vi "Delete Scale.vi"(8 "error in":errorcluster, 10 "Index":i32, 11 "references":T1) -> (0 "error out":errorcluster)   [LabVIEW 2014, in "Scaling editor node.lvclass"]
uses:
  Scaling editor node.lvclass
  <vilib>/NI/DCAF/Tag Editor Core/Table API/Table Manager/object ref.ctl
  <vilib>/NI/DCAF/Tag Editor Core/Configuration Editor/Classes/Engine Parent/Engine Parent Editor Node.lvclass
  <vilib>/NI/DCAF/Tag Editor Core/Configuration Editor/Classes/Module editor node/module editor node.lvclass
  module/configuration/Scaling configuration.lvclass
  <vilib>/NI/Configuration Framework/serializable configuration/NISE_CEF_serializable configuration.lvclass/NISE_CEF_serializable configuration.ctl
  <vilib>/Utility/LVClass/Get LV Class Name.vi
  <vilib>/NI/Configuration Framework/error generator/NISE_error generator.vi
  <vilib>/NI/Tag Bus Module Framework/channel/TBM channel.lvclass
  <vilib>/NI/Configuration Framework/serializable configuration/NISE_CEF_serializable configuration.lvclass
  <vilib>/NI/Module Execution Interface/Engine Configuration/engine configuration.lvclass
  <vilib>/NI/DCAF/Tag Editor Core/Table API/Table Manager/Table Manager.lvclass
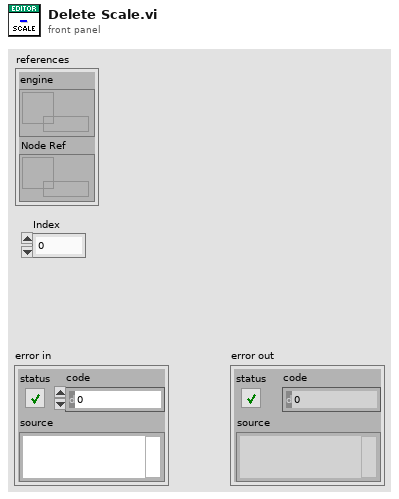
[diagram p1: front panel]
types:
  T1 = typedef "Table Manager.lvlib/Table Manager.lvclass/object ref.ctl" = cluster{"engine":refnum<data-value>, "Node Ref":refnum<data-value>}
  T2 = typedef "Scaling configuration.lvclass/scale data types.ctl" = enum16{"Double", "Single", "I64", "I32", "I16", "I8", "U64", "U32", "U16", "U8", "Boolean"}
  T3 = cluster{"input channel":refnum<class "TBM channel.lvclass">, "output channel":refnum<class "TBM channel.lvclass">, "input data type":T2, "output data type":T2}[]
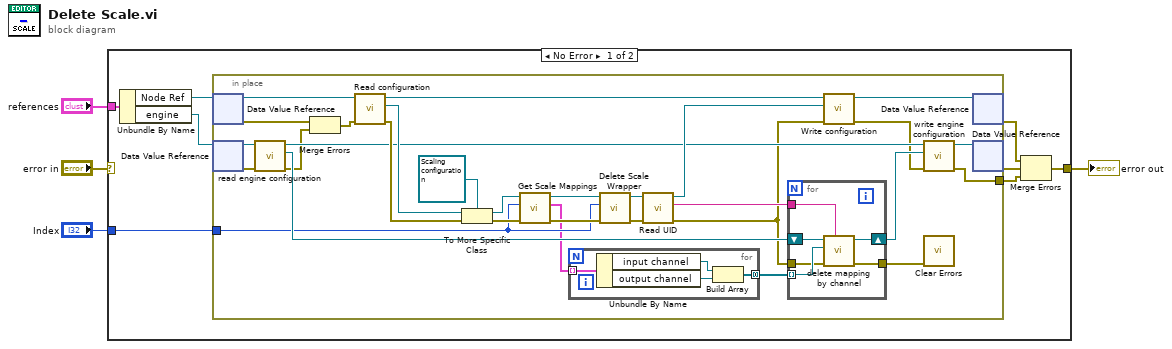
[diagram p0: block diagram]
diagram:
  n1 = case shown="No Error" "error in" {
    selector: "error in" -> [_ w53]
    tunnel: [w6 w53] -> w2
    tunnel: "Index" -> [w11 _]
    tunnel: "references" -> [w5 _]
    frame No Error {
      n2 = Unbundle By Name(w5) -> ("Node Ref"=w12:refnum<data-value>, "engine"=w10:refnum<data-value>)
      n3 = in-place {
        in-place-border: [w14] -> w7
        in-place-border: w11 -> [w19]
        n4 = in-place-dvr #1(w12) -> (w41:refnum<class "module editor node.lvclass">, w26:errorcluster)
        n5 = in-place-dvr #2(w10) -> (w36:refnum<class "Engine Parent Editor Node.lvclass">, w27:errorcluster)
        n6 = call <vilib>:"read engine configuration.vi"("error in"=w27, "Engine Parent Editor Node in"=w36) -> ("error out"=w25:errorcluster, "engine configuration"=w31:refnum<class "engine configuration.lvclass">, "Engine Parent Editor Node out"=w28:refnum<class "Engine Parent Editor Node.lvclass">)  [unwired: 7 in]
        n7 = Merge Errors(w26, w25) -> (w24:errorcluster)
        n8 = call-dynamic "Read configuration.vi"("error in"=w24, "NISE_CEF_serializable node in"=w41) -> ("error out"=w37:errorcluster, "configuration"=w40:refnum<class "NISE_CEF_serializable configuration.lvclass">, "NISE_CEF_serializable node out"=w42:refnum<class "module editor node.lvclass">)  [unwired: 7 in]
        n9 = To More Specific Class(target class=refnum<class "Scaling configuration.lvclass"> refnum ("Scaling configuration"), reference=w40, error in=w37) -> (specific class reference=w22:refnum<class "Scaling configuration.lvclass">, error out=w21:errorcluster)
        n10 = call "Get Scale Mappings.vi"("error in (no error)"=w21, "index"=w19, "Scaling configuration in"=w22) -> ("error out"=w20:errorcluster, "mappings"=w17:T3, "Scaling configuration out"=w18:refnum<class "Scaling configuration.lvclass">)  [unwired: 6 in]
        n11 = for {
          tunnel: w17 -> [w46] mode=indexing
          tunnel: [w43] -> w16 mode=concatenating
          n12 = Unbundle By Name(w46) -> ("input channel"=w45:refnum<class "TBM channel.lvclass">, "output channel"=w44:refnum<class "TBM channel.lvclass">)
          n13 = Build Array(w45, w44) -> (w43:refnum<class "TBM channel.lvclass">[])
        }
        n14 = call "Delete Scale Wrapper.vi"("error in"=w20, "index"=w19, "Scaling configuration in"=w18) -> ("error out"=w33:errorcluster, "Scaling configuration out"=w34:refnum<class "Scaling configuration.lvclass">)  [unwired: 7 in]
        n15 = call <vilib>:"Read UID.vi"("error in"=w33, "configuration in"=w34) -> ("error out"=w23:errorcluster, "instance id"=w29:string, "configuration out"=w32:refnum<class "Scaling configuration.lvclass">)  [unwired: 7 in]
        n16 = for {
          tunnel: w16 -> [w52] mode=indexing
          shift-right: [w49] -> w30
          shift-left: w31 -> [w50]
          tunnel: w29 -> [w48]
          tunnel: w23 -> [w51]
          tunnel: [w47] -> w13
          n17 = call <vilib>:"delete mapping by channel.vi"("owner ID"=w48, "error in"=w51, "channel"=w52, "engine configuration in"=w50) -> ("error out"=w47:errorcluster, "engine configuration out"=w49:refnum<class "engine configuration.lvclass">)  [unwired: 6 in]
        }
        n18 = call-dynamic "Write configuration.vi"("error in"=w23, "configuration"=w32, "NISE_CEF_serializable node in"=w42) -> ("error out"=w15:errorcluster, "NISE_CEF_serializable node out"=w39:refnum<class "module editor node.lvclass">)  [unwired: 7 in]
        n19 = call <vilib>:"write engine configuration.vi"("error in"=w15, "engine configuration"=w30, "Engine Parent Editor Node in"=w28) -> ("error out"=w14:errorcluster, "Engine Parent Editor Node out"=w35:refnum<class "Engine Parent Editor Node.lvclass">)  [unwired: 7 in]
        n20 = call <vilib>:"Clear Errors.vi"("error in (no error)"=w13) -> ()  [unwired: 5 in, 2 out]
        n21 = in-place-dvr #1(w39) -> (w9:errorcluster)  [unwired: 1 out]
        n22 = in-place-dvr #2(w35) -> (w8:errorcluster)  [unwired: 1 out]
      }
      n23 = Merge Errors(w9, w8, w7) -> (w6:errorcluster)
    }
    frame Error {
    }
  }
  "error out" <- w2
